vi "Filter_Evaluator.vi"(7 "Headers":string[](array[string])=["Packet_Number", "Timestamp", "Source", "Destination", "Protocol", "Length", "Data"], 8 "Error":errorcluster, 9 "Comparators":T1(array[cluster]), 10 "Boolean Connectors":string[](array[string])=["AND", "OR"], 11 "Prefiltered Data":string[][](array[string])=array1500x7[10500 elements]) -> (0 "Error Out":errorcluster, 2 "Filtered Array":string[][](array[string]), 3 "Prefiltered Data":string[][](array[string]))   [LabVIEW 2025, in "Table_Filtering.lvlib"]
uses:
  Table_Filtering.lvlib
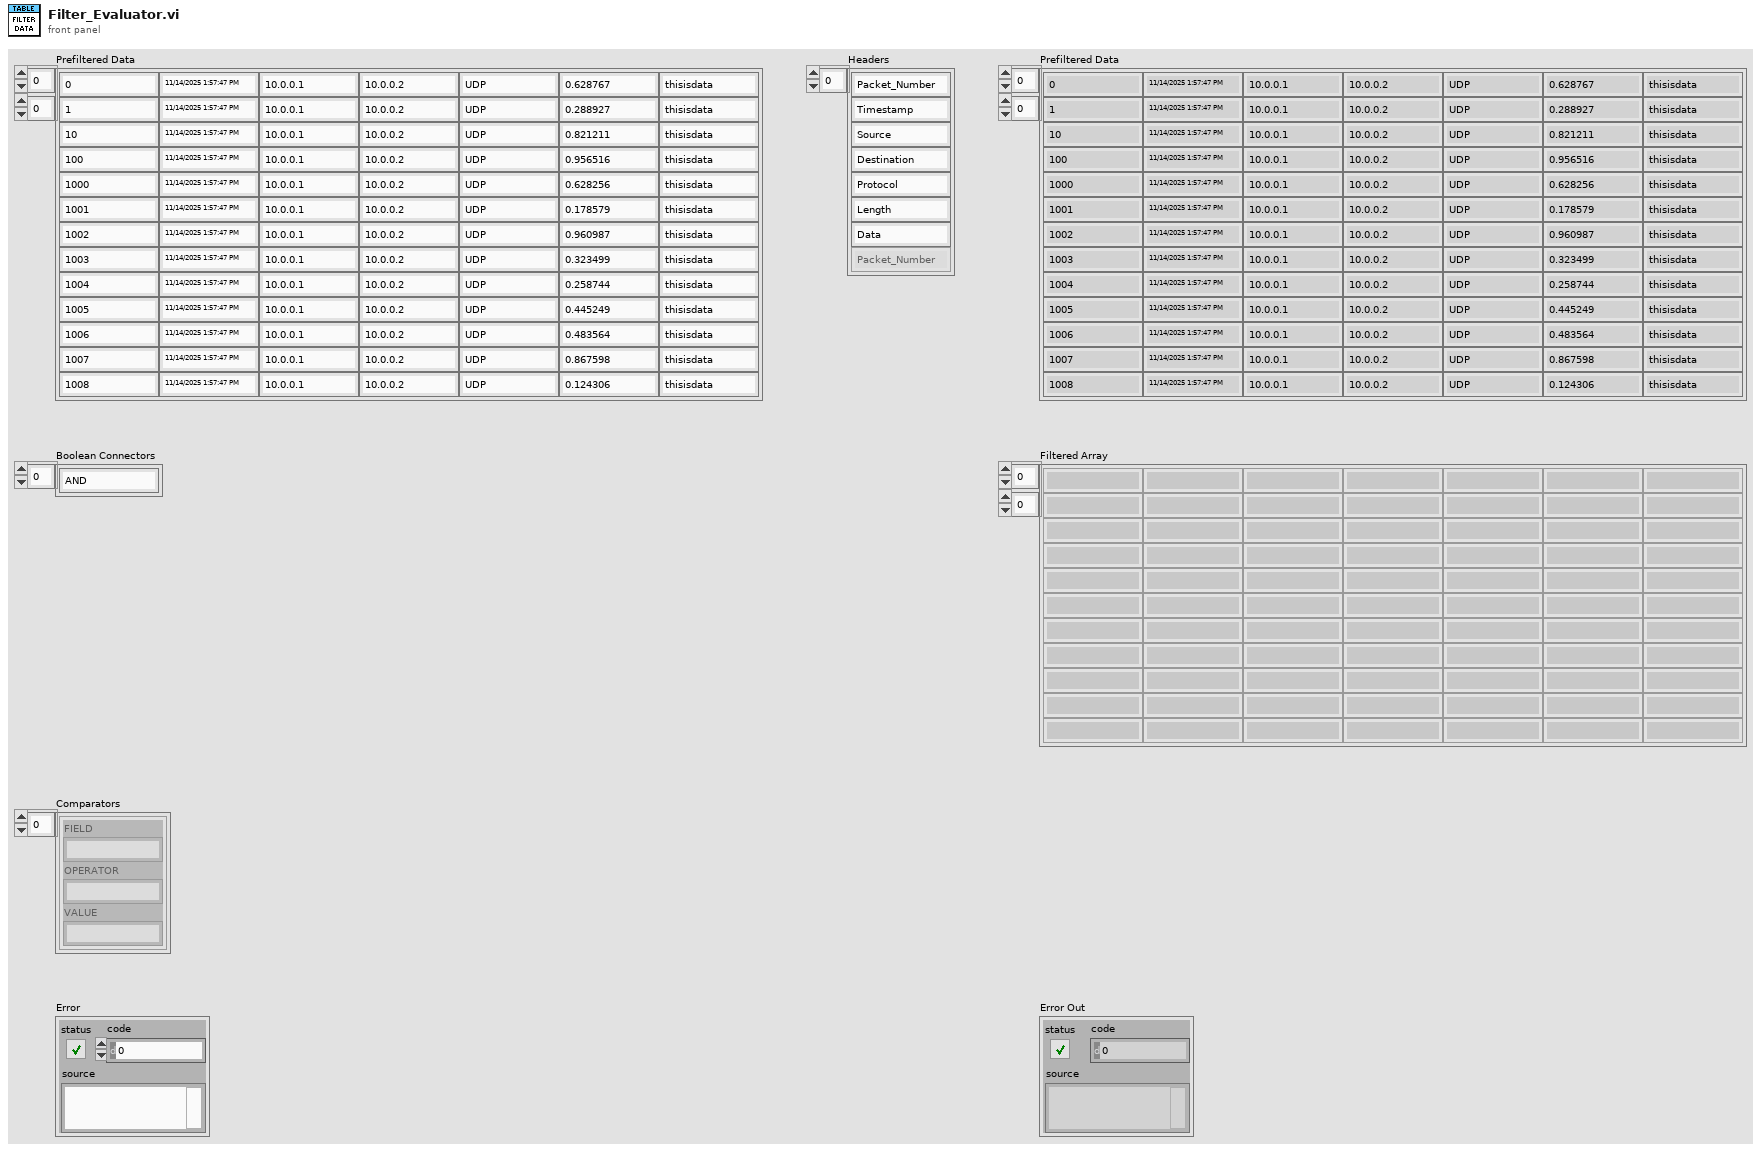
[diagram p1: front panel]
types:
  T1 = cluster{"FIELD":string, "OPERATOR":string, "VALUE":string}[]
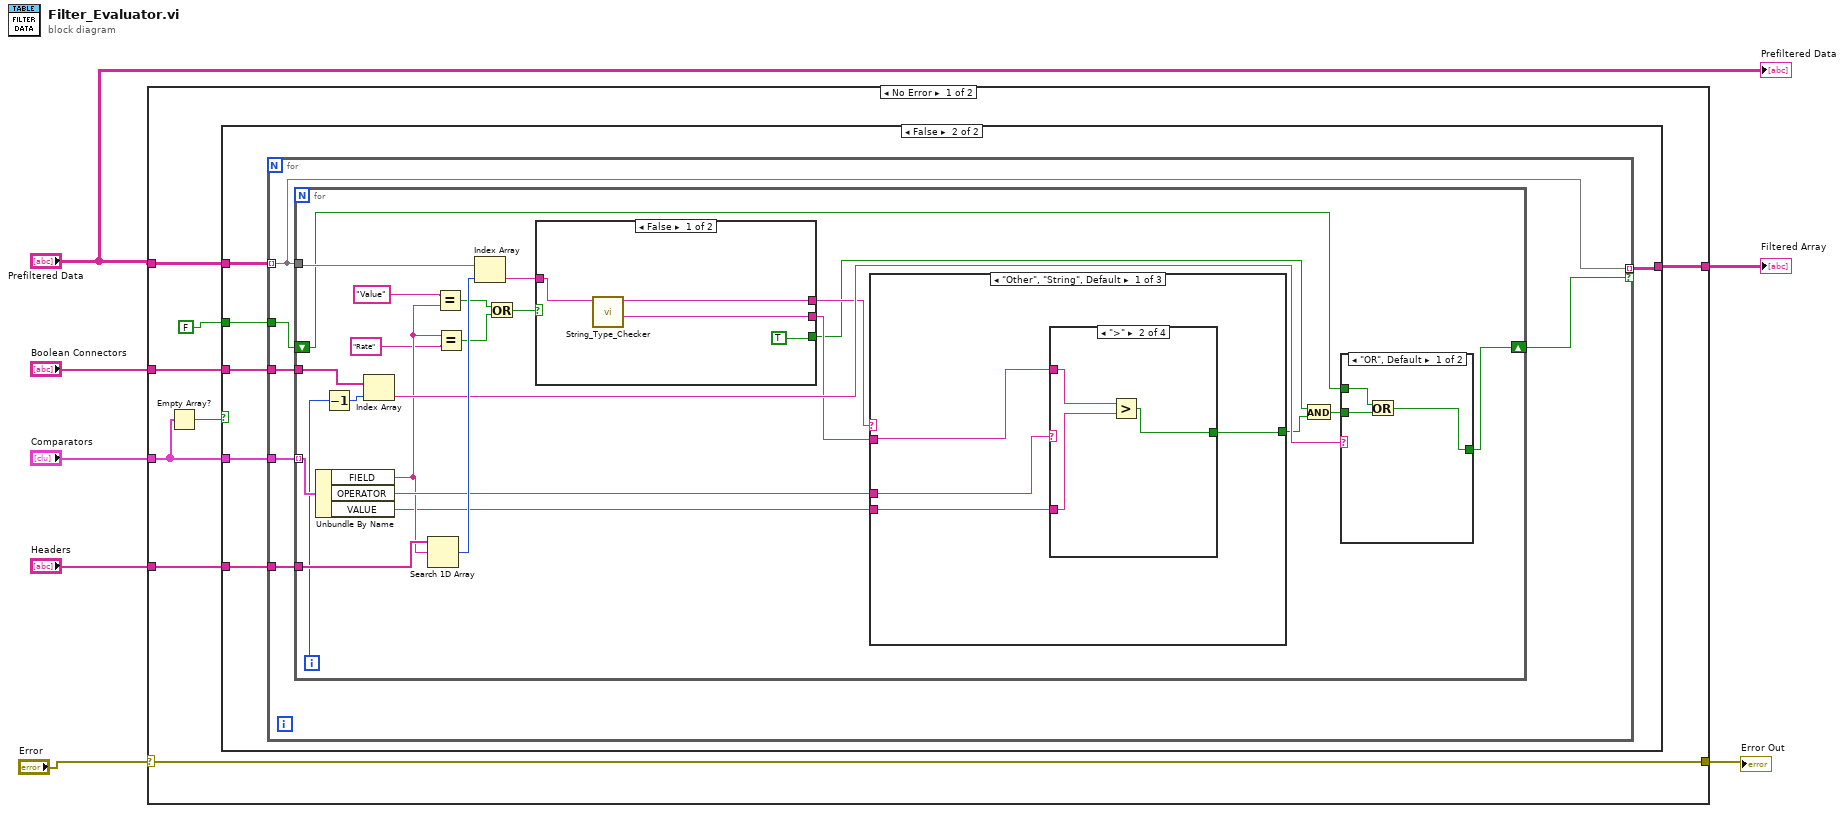
[diagram p0: block diagram]
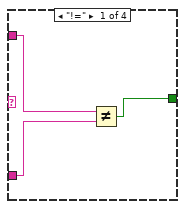
[diagram p3: hidden frame]
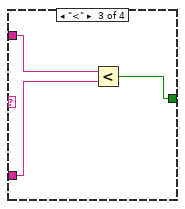
[diagram p4: hidden frame]
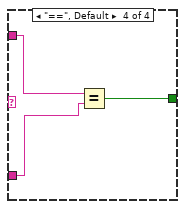
[diagram p5: hidden frame]
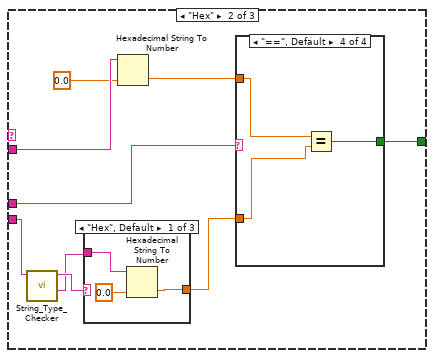
[diagram p6: hidden frame]
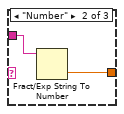
[diagram p7: hidden frame]
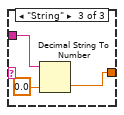
[diagram p8: hidden frame]
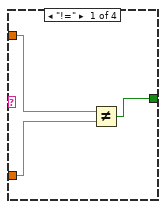
[diagram p9: hidden frame]
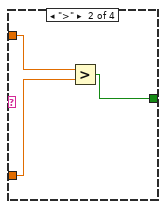
[diagram p10: hidden frame]
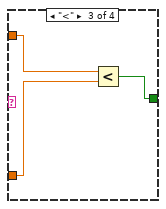
[diagram p11: hidden frame]
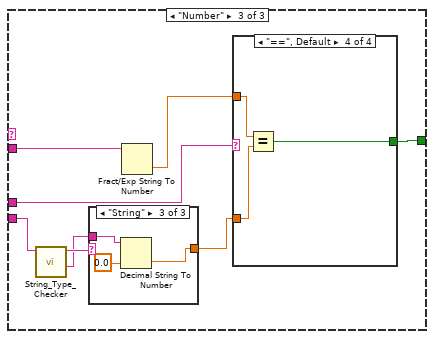
[diagram p12: hidden frame]
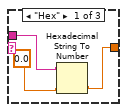
[diagram p13: hidden frame]
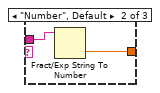
[diagram p14: hidden frame]
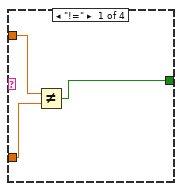
[diagram p15: hidden frame]
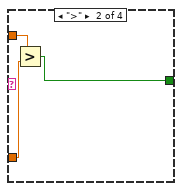
[diagram p16: hidden frame]
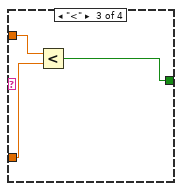
[diagram p17: hidden frame]
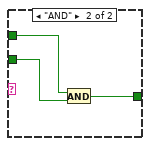
[diagram p18: hidden frame]
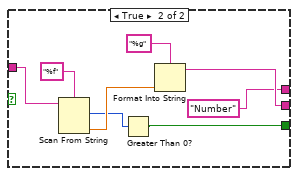
[diagram p19: hidden frame]
diagram:
  n1 = case shown="No Error" "Error" {
    selector: "Error" -> [w11 w144]
    tunnel: "Headers" -> [w15 _]
    tunnel: "Boolean Connectors" -> [w14 _]
    tunnel: "Comparators" -> [w8 _]
    tunnel: "Prefiltered Data" -> [w13 _]
    tunnel: [w12 _] -> w7
    tunnel: [w11 w144] -> w2
    frame No Error {
      n2 = Empty Array?(array=w8) -> (empty?=w9:bool)
      n3 = case shown="False" w9 {
        tunnel: w15 -> [_ w22]
        tunnel: FALSE -> [_ w21]
        tunnel: w14 -> [_ w20]
        tunnel: w8 -> [_ w19]
        tunnel: w13 -> [w16 w18]
        tunnel: [w16 w17] -> w12
        frame True {
        }
        frame False {
          n4 = for {
            tunnel: w22 -> [w28]
            tunnel: w19 -> [w27]
            tunnel: w18 -> [w23] mode=indexing
            tunnel: w21 -> [w26]
            tunnel: w20 -> [w25]
            tunnel: [w23] -> w17 mode=indexing if=w24
            n5 = for {
              tunnel: w28 -> [w50]
              tunnel: w27 -> [w52] mode=indexing
              tunnel: w23 -> [w51]
              shift-right: [w44] -> w24
              shift-left: w26 -> [w45]
              tunnel: w25 -> [w48]
              i -> [w46]
              n6 = Unbundle By Name(w52) -> ("FIELD"=w38:string, "OPERATOR"=w43:string, "VALUE"=w32:string)
              n7 = Decrement(x=w46) -> (x-1=w47:i32)
              n8 = Index Array(array=w48, index=w47) -> (element=w42:string)
              n9 = Search 1D Array(1D array=w50, element=w38) -> (index of element=w49:i32)  [unwired: 1 in]
              n10 = Equal?(x="Value", y=w38) -> (x = y?=w40:bool)
              n11 = Equal?(x=w38, y="Rate") -> (x = y?=w39:bool)
              n12 = Index Array(array=w51, index=w49) -> (element=w35:string)
              n13 = Or(x=w40, y=w39) -> (x .or. y?=w41:bool)
              n14 = case shown="False" w41 {
                tunnel: w35 -> [w135 w143]
                tunnel: [w134 w139] -> w34
                tunnel: [w133 "Number" ("Type")] -> w33
                tunnel: [TRUE w136] -> w30
                frame False {
                  n15 = call "String_Type_Checker.vi"("String"=w135) -> ("Number"=w134:string, "Type"=w133:string)  [unwired: 9 in]
                }
                frame True {
                  n16 = Scan From String(format string="%f", input string=w143) -> (offset past scan=w137:u32, output 1=w141:dbl)  [unwired: 3 in, 2 out]
                  n17 = Greater Than 0?(x=w137) -> (x > 0?=w136:bool)
                  n18 = Format Into String(format string="%g", w141) -> (resulting string=w139:string)  [unwired: 2 in, 1 out]
                }
              }
              n19 = case shown="\"Other\", \"String\", Default" w33 {
                tunnel: w34 -> [w56 w77 w105]
                tunnel: w32 -> [w53 w72 w101]
                tunnel: w43 -> [w55 w75 w104]
                tunnel: [w54 w74 w103] -> w31
                frame "Other", "String", Default {
                  n20 = case shown="\">\"" w55 {
                    tunnel: w56 -> [w58 w62 w65 w66]
                    tunnel: w53 -> [w57 w61 w64 w68]
                    tunnel: [w59 w60 w63 w67] -> w54
                    frame "!=" {
                      n21 = Not Equal?(x=w58, y=w57) -> (x != y?=w59:bool)
                    }
                    frame ">" {
                      n22 = Greater?(x=w62, y=w61) -> (0:w60:bool)
                    }
                    frame "<" {
                      n23 = Less?(x=w65, y=w64) -> (x < y?=w63:bool)
                    }
                    frame "==", Default {
                      n24 = Equal?(x=w66, y=w68) -> (x = y?=w67:bool)
                    }
                  }
                }
                frame "Hex" {
                  n25 = call "String_Type_Checker.vi"("String"=w72) -> ("Number"=w69:string, "Type"=w70:string)  [unwired: 9 in]
                  n26 = case shown="\"Hex\", Default" w70 {
                    tunnel: [w78 w82 w85] -> w73
                    tunnel: w69 -> [w80 w81 w83]
                    frame "Hex", Default {
                      n27 = Hexadecimal String To Number(string=w80, default (0uL)=0.0) -> (number=w78:dbl)  [unwired: 1 in, 1 out]
                    }
                    frame "Number" {
                      n28 = Fract/Exp String To Number(string=w81) -> (number=w82:dbl)  [unwired: 3 in, 1 out]
                    }
                    frame "String" {
                      n29 = Decimal String To Number(string=w83, default (0L)=0.0) -> (number=w85:dbl)  [unwired: 1 in, 1 out]
                    }
                  }
                  n30 = Hexadecimal String To Number(string=w77, default (0uL)=0.0) -> (number=w76:dbl)  [unwired: 1 in, 1 out]
                  n31 = case shown="\"==\", Default" w75 {
                    tunnel: w76 -> [w87 w91 w94 w95]
                    tunnel: w73 -> [w86 w90 w93 w97]
                    tunnel: [w88 w89 w92 w96] -> w74
                    frame "!=" {
                      n32 = Not Equal?(x=w87, y=w86) -> (x != y?=w88:bool)
                    }
                    frame ">" {
                      n33 = Greater?(x=w91, y=w90) -> (0:w89:bool)
                    }
                    frame "<" {
                      n34 = Less?(x=w94, y=w93) -> (x < y?=w92:bool)
                    }
                    frame "==", Default {
                      n35 = Equal?(x=w95, y=w97) -> (x = y?=w96:bool)
                    }
                  }
                }
                frame "Number" {
                  n36 = call "String_Type_Checker.vi"("String"=w101) -> ("Number"=w99:string, "Type"=w100:string)  [unwired: 9 in]
                  n37 = case shown="\"String\"" w100 {
                    tunnel: [w106 w110 w113] -> w98
                    tunnel: w99 -> [w108 w109 w111]
                    frame "Hex" {
                      n38 = Hexadecimal String To Number(string=w108, default (0uL)=0.0) -> (number=w106:dbl)  [unwired: 1 in, 1 out]
                    }
                    frame "Number", Default {
                      n39 = Fract/Exp String To Number(string=w109) -> (number=w110:dbl)  [unwired: 3 in, 1 out]
                    }
                    frame "String" {
                      n40 = Decimal String To Number(string=w111, default (0L)=0.0) -> (number=w113:dbl)  [unwired: 1 in, 1 out]
                    }
                  }
                  n41 = Fract/Exp String To Number(string=w105) -> (number=w102:dbl)  [unwired: 3 in, 1 out]
                  n42 = case shown="\"==\", Default" w104 {
                    tunnel: w98 -> [w115 w119 w122 w125]
                    tunnel: [w116 w118 w121 w124] -> w103
                    tunnel: w102 -> [w114 w117 w120 w123]
                    frame "!=" {
                      n43 = Not Equal?(x=w114, y=w115) -> (x != y?=w116:bool)
                    }
                    frame ">" {
                      n44 = Greater?(x=w117, y=w119) -> (0:w118:bool)
                    }
                    frame "<" {
                      n45 = Less?(x=w120, y=w122) -> (x < y?=w121:bool)
                    }
                    frame "==", Default {
                      n46 = Equal?(x=w123, y=w125) -> (x = y?=w124:bool)
                    }
                  }
                }
              }
              n47 = And(x=w30, y=w31) -> (x .and. y?=w29:bool)
              n48 = case shown="\"OR\", Default" w42 {
                tunnel: w45 -> [w127 w131]
                tunnel: [w128 w130] -> w44
                tunnel: w29 -> [w126 w129]
                frame "OR", Default {
                  n49 = Or(x=w127, y=w126) -> (x .or. y?=w128:bool)
                }
                frame "AND" {
                  n50 = And(x=w131, y=w129) -> (x .and. y?=w130:bool)
                }
              }
            }
          }
        }
      }
    }
    frame Error {
    }
  }
  "Filtered Array" <- w7
  "Error Out" <- w2
  "Prefiltered Data" <- "Prefiltered Data"
